vi "Get Start Stop Threshold.vi"(6 "nStopThreshold":i32, 7 "nStartThreshold":i32, 8 "error in (no error)":errorcluster caption="错误输入（无错误）", 9 "nChannel":i32, 10 "nBoard":i32, 11 "nDevId":i32) -> (0 "error out":errorcluster caption="错误输出", 3 "function return":i32, 4 "nStopThreshold out":i32, 5 "nStartThreshold out":i32)   [LabVIEW 2017, in "smncsftmt.lvlib"]
doc: "__declspec(dllexport) int GetStartStopThreshold(int nDevId, int nBoard, int nChannel, int* nStartThreshold, int* nStopThreshold);"
uses:
  smncsftmt.lvlib
  smncsftmt.dll
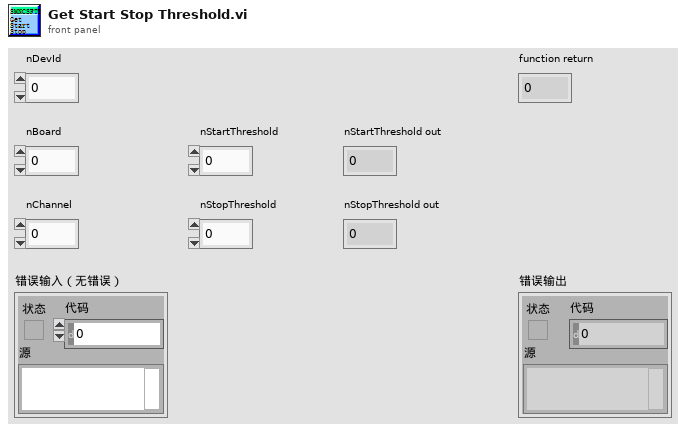
[diagram p1: front panel]
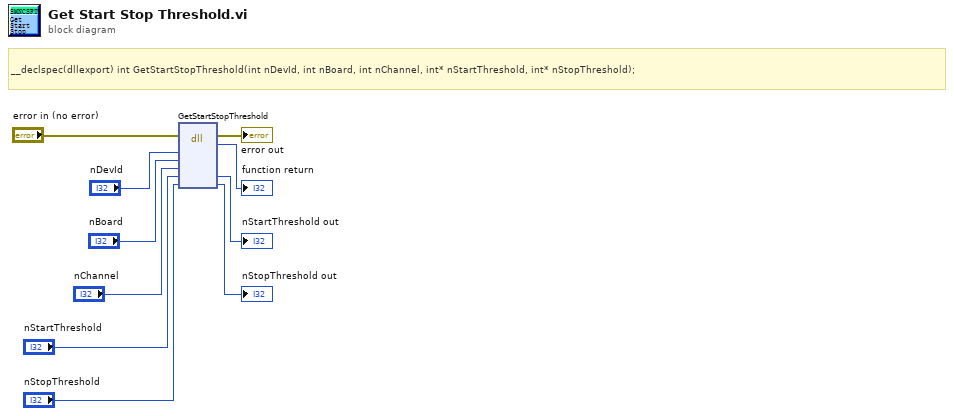
[diagram p0: block diagram]
diagram:
  # "__declspec(dllexport) int GetStartStopThreshold(int nDevId, int nBoard, int nChannel, int* nStartThreshold, int* nStopThreshold);"
  n1 = dll-call lib="PTH2oabs CUsersaDesktop\nLABVIEW范例National InstrumentsLabVIEW 2017user.lib\tsmncsftmtsmncsftmt.*" fn="GetStartStopThreshold"(error in="error in (no error)", "nDevId"="nDevId", "nBoard"="nBoard", "nChannel"="nChannel", "nStartThreshold"="nStartThreshold", "nStopThreshold"="nStopThreshold") -> (error out=→"error out":errorcluster, →"function return":i32, "nStartThreshold"=→"nStartThreshold out":i32, "nStopThreshold"=→"nStopThreshold out":i32)  [unwired: 5 in, 1 out]
